vi "Host Main.vi"() -> ()   [LabVIEW 2015]
doc: "This application launches and executes the Tag Bus Data framework configuration for the specified target alias. This is a simple example of the framework API functions, but may also be a suitable starting point for a Host UI or Thick Client that is running a local version of the framework."
uses:
  <vilib>/NI/Module Execution Interface/Engine Runtime/Execution States.ctl
  <vilib>/NI/Module Execution Interface/Engine Runtime/Fault.ctl
  <vilib>/NI/Tag Bus Module Framework/runtime/error classification.ctl
  <vilib>/NI/Current Value Table/DataTypes/I32_Read.vi
  <vilib>/NI/Current Value Table/DataTypes/I32_Write.vi
  <vilib>/NI/Current Value Table/Type to Enum.vi
  <vilib>/NI/Current Value Table/DataTypes/I32_Type To Enum.vi
  <vilib>/NI/Current Value Table/FGVs/CVT Globals.vi
  <vilib>/NI/Current Value Table/FGVs/Tag Memory.vi
  <vilib>/NI/Current Value Table/Memory Block.vi
  <vilib>/NI/Current Value Table/DataTypes/I32_Memory Block.vi
  <vilib>/NI/Module Execution Interface/Engine Runtime/Engine Runtime Interface.lvclass
  <vilib>/NI/DCAF/Tag Editor Core/Framework Configuration Classes/target runtime/PL_Target Runtime.lvclass
  <vilib>/NI/Current Value Table/Current Value Table.lvlib
  <vilib>/NI/Tag Bus Module Framework/runtime/TBM module execution interface.lvclass
panel:
  in  "Boolean":bool=TRUE
  out "Value":i32
  in  "I32 Control":i32
  in  "configuration file path":path=path "/home/lvuser/FPGATestConfig.pcfg"
  in  "target alias":string="cRIO"
  out "engine status":T4(array[cluster])
  in  "stop":bool
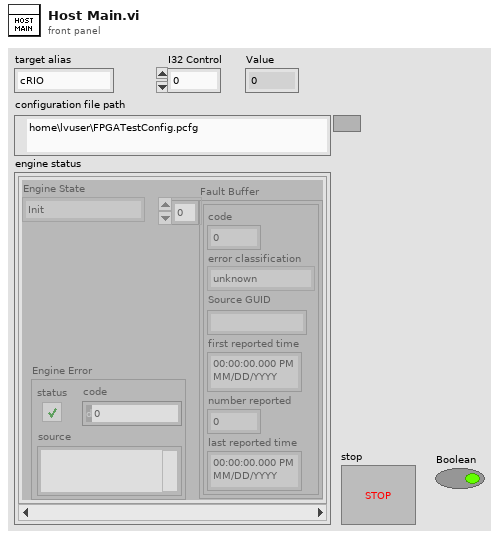
[diagram p1: front panel]
types:
  T1 = typedef "Engine Runtime Interface.lvclass/Execution States.ctl" = enum16{"Init", "Pre-Operational", "Safe-Operational", "Operational", "Stopped"}
  T2 = typedef "Engine Runtime Interface.lvclass/Fault.ctl" = cluster{"code":i32, "error classification":T3, "Source GUID":string, "first reported time":timestamp, "number reported":u32, "last reported time":timestamp}
  T3 = typedef "TBM module execution interface.lvclass/error classification.ctl" = enum16{"unknown", "none", "trivial", "recoverable", "critical"}
  T4 = cluster{"Engine State":T1, "Fault Buffer":T2[], "Engine Error":errorcluster}[]
  T5 = cluster{"Engine State":T1, "faults":T2[], "Engine Error":errorcluster}
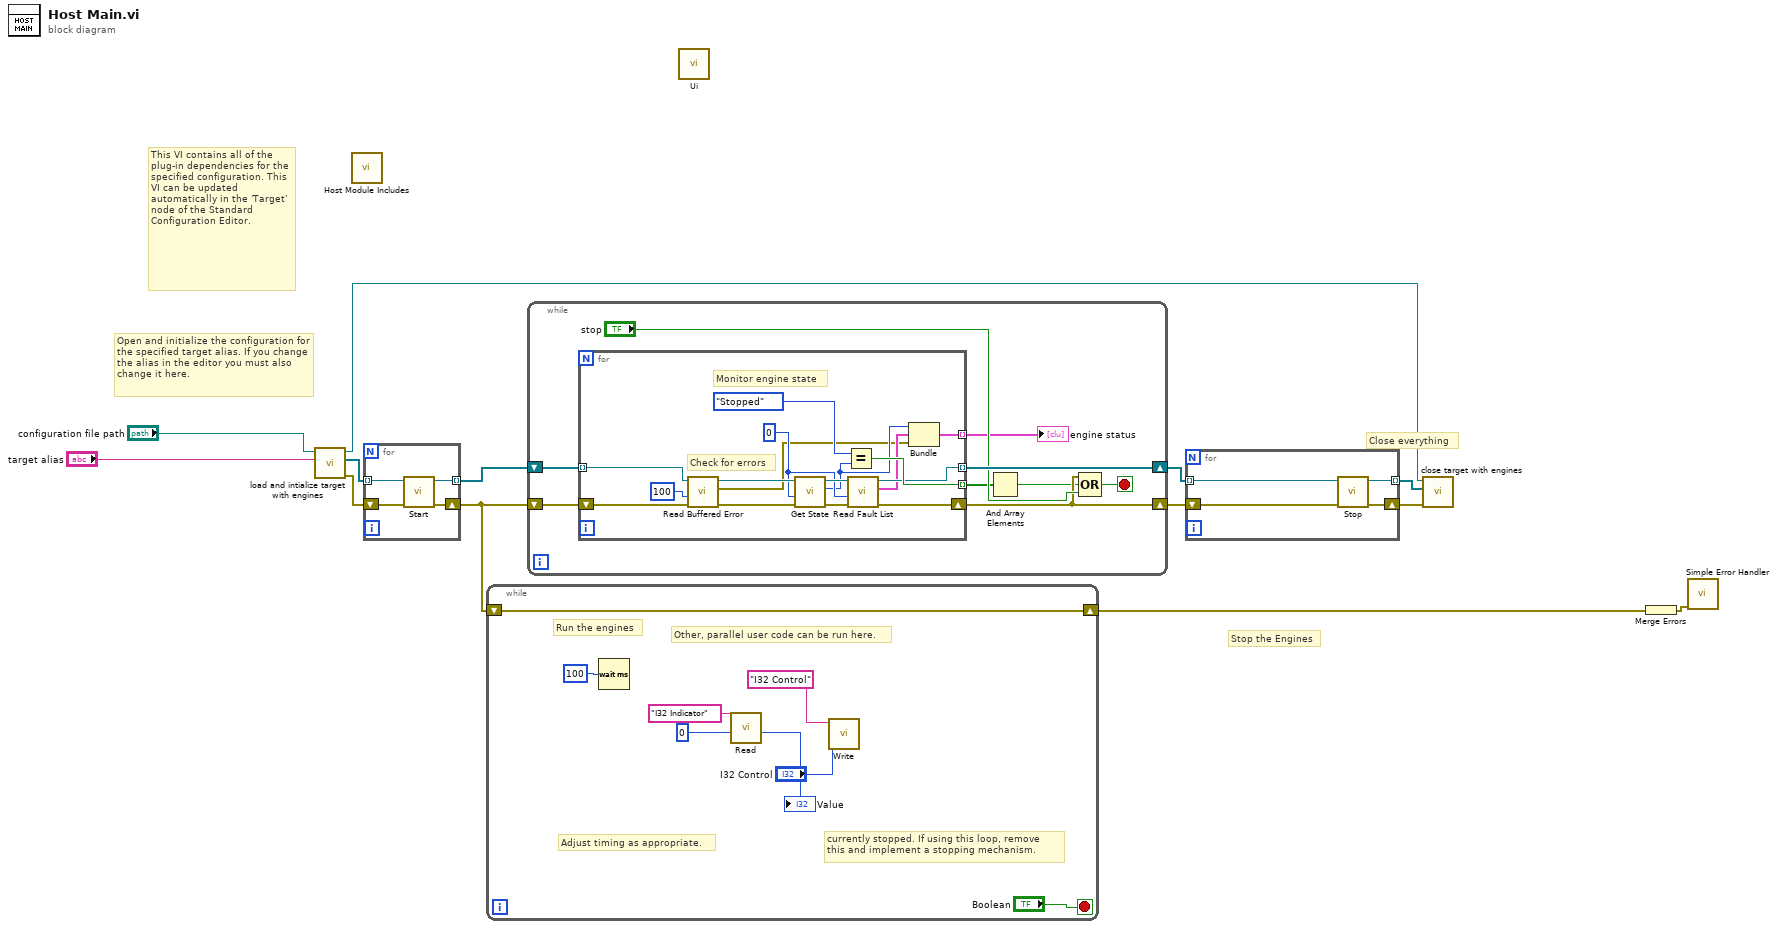
[diagram p0: block diagram]
diagram:
  # "Open and initialize the configuration for the specified target alias. If you change the alias in the editor you must also change it here."
  # "Close everything"
  # "Stop the Engines"
  # "This VI contains all of the plug-in dependencies for the specified configuration. This VI can be updated automatically in the 'Target' node of the Standard Configuration Editor."
  # "Run the engines"
  n1 = call <vilib>:"load and intialize target with engines.vi"("target alias"="target alias", "file path"="configuration file path") -> ("error out"=w10:errorcluster, "engine runtime interfaces"=w9:refnum<class "Engine Runtime Interface.lvclass">[], "target runtime"=w6:refnum<class "PL_Target Runtime.lvclass">)  [unwired: 7 in]
  n2 = call "Host Module Includes.vi"() -> ()  [unwired: 12 in]
  n3 = for {
    tunnel: [w17] -> w13 mode=indexing
    tunnel: w9 -> [w14] mode=indexing
    shift-right: [w16] -> w3
    shift-left: w10 -> [w15]
    n4 = call-dynamic "Start.vi"("error in"=w15, "Engine Runtime Interface in"=w14) -> ("error out"=w16:errorcluster, "Engine Runtime Interface out"=w17:refnum<class "Engine Runtime Interface.lvclass">)  [unwired: 8 in]
  }
  n5 = while {
    shift-right: [w23] -> w2
    shift-left: w3 -> [w23]
    stop <- "Boolean" stop-if-true
    # "currently stopped. If using this loop, remove \nthis and implement a stopping mechanism."
    # "Adjust timing as appropriate."
    # "Other, parallel user code can be run here."
    n6 = Wait (ms)(milliseconds to wait=u32 100) -> ()  [unwired: 1 out]
    n7 = call-poly <vilib>:"Read.vi"("Default"=0, "Tag Name"="I32 Indicator") -> ("Value"=→"Value":i32)  [unwired: 8 in, 1 out]
    n8 = call-poly <vilib>:"Write.vi"("Value"="I32 Control", "Tag Name"="I32 Control") -> ()  [unwired: 9 in, 1 out]
  }
  n9 = while {
    shift-right: [w32] -> w12
    shift-left: w13 -> [w34]
    shift-right: [w29] -> w11
    shift-left: w3 -> [w33]
    stop <- w30 stop-if-true
    n10 = for {
      tunnel: w34 -> [w50] mode=indexing
      tunnel: [w41] -> w32 mode=indexing
      tunnel: [w45] -> w27 mode=indexing
      shift-right: [w40] -> w29
      shift-left: w33 -> [w49]
      tunnel: [w35] -> w28 mode=indexing
      w39 = 0 ("timeout (-1)")
      # "Monitor engine state"
      # "Check for errors"
      n11 = call-dynamic "Read Buffered Error.vi"("error in"=w49, "timeout in ms (0)"=100, "Engine Runtime Interface in"=w50) -> ("error out"=w47:errorcluster, "Engine Error"=w36:errorcluster, "Engine Runtime Interface out"=w48:refnum<class "Engine Runtime Interface.lvclass">)  [unwired: 6 in]
      n12 = call-dynamic "Get State.vi"("error in"=w47, "timeout (-1)"=w39, "Engine Runtime Interface in"=w48) -> ("error out"=w43:errorcluster, "Engine State"=w38:T1, "Engine Runtime Interface out"=w42:refnum<class "Engine Runtime Interface.lvclass">)  [unwired: 6 in]
      n13 = Equal?(x=Execution_States."Stopped" ("Engine State"), y=w38) -> (x = y?=w45:bool)
      n14 = call-dynamic "Read Fault List.vi"("error in"=w43, "timeout (-1)"=w39, "Engine Runtime Interface in"=w42) -> ("error out"=w40:errorcluster, "faults"=w37:T2[], "Engine Runtime Interface out"=w41:refnum<class "Engine Runtime Interface.lvclass">)  [unwired: 6 in]
      n15 = Bundle("Engine State"=w38, "faults"=w37, "Engine Error"=w36) -> (w35:T5)  [unwired: 1 in]
    }
    "engine status" <- w28
    n16 = And Array Elements(Boolean array=w27) -> (logical AND=w26:bool)
    n17 = Compound Arithmetic op=OR(w29, w26, "stop") -> (w30:bool)
  }
  n18 = call "Ui.vi"() -> ()  [unwired: 12 in]
  n19 = for {
    tunnel: w12 -> [w54] mode=indexing
    shift-right: [w51] -> w5
    shift-left: w11 -> [w53]
    tunnel: [w52] -> w7 mode=indexing
    n20 = call-dynamic "Stop.vi"("error in"=w53, "Engine Runtime Interface in"=w54) -> ("error out"=w51:errorcluster, "Engine Runtime Interface out"=w52:refnum<class "Engine Runtime Interface.lvclass">)  [unwired: 8 in]
  }
  n21 = call <vilib>:"close target with engines.vi"("error in"=w5, "Engine Runtime Interfaces"=w7, "Target Runtime"=w6) -> ()  [unwired: 8 in, 1 out]
  n22 = Merge Errors(w2) -> (w1:errorcluster)
  n23 = call <vilib>:"Simple Error Handler.vi"("error in (no error)"=w1) -> ()  [unwired: 4 in, 5 out]
